vi "OnTrak_ADU_Write.vi"(2 "iTimeout":u32=200, 3 "Set Relay":i32=4 min=0 max=4 step=1, 4 "Output":u8 step=1 format="%x", 5 "psSerialNumber":string="E06002") -> (0 "OutPutNumber":i32 format="%x", 1 "error out":errorcluster)   [LabVIEW 2013]
uses:
  AduHid.dll
panel:
  out "OutPutStr":string="PK"
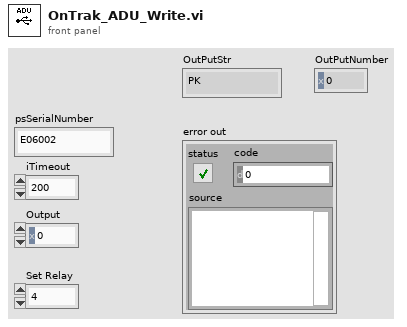
[diagram p1: front panel]
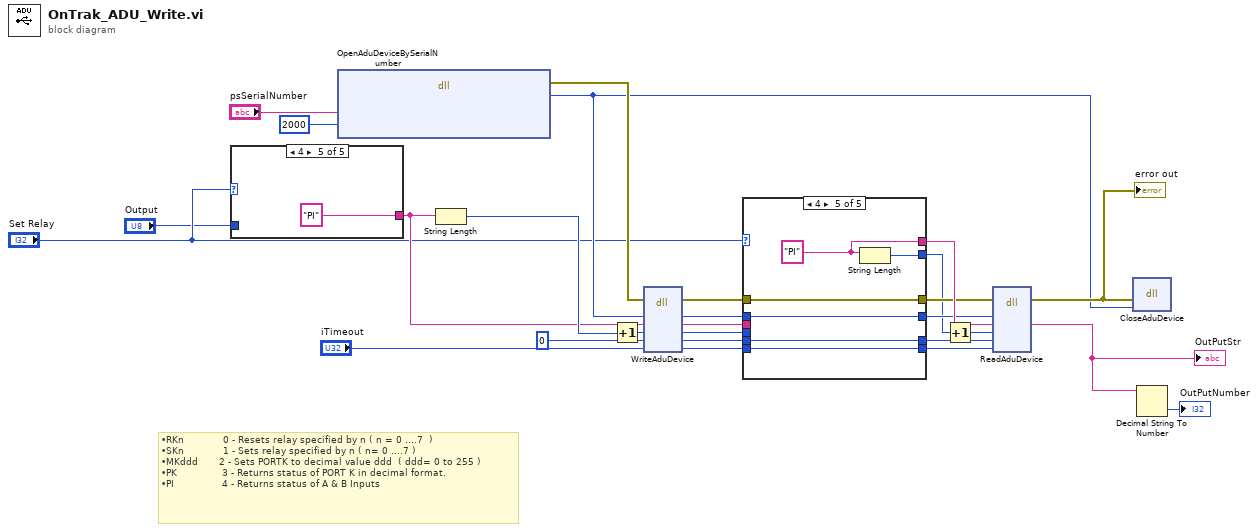
[diagram p0: block diagram]
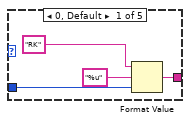
[diagram p2: hidden frame]
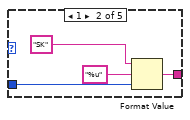
[diagram p3: hidden frame]
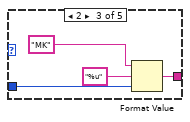
[diagram p4: hidden frame]
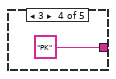
[diagram p5: hidden frame]
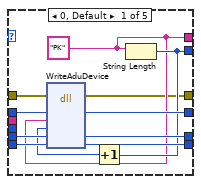
[diagram p6: hidden frame]
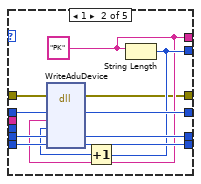
[diagram p7: hidden frame]
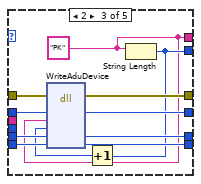
[diagram p8: hidden frame]
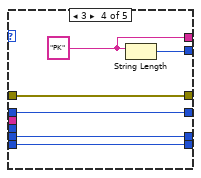
[diagram p9: hidden frame]
diagram:
  # "•RKn             0 - Resets relay specified by n ( n = 0 ....7  ) \n•SKn             1 - Sets relay specified by n ( n= 0 ....7 )\n•MKddd       2 - Sets PORTK to decimal value ddd  ( ddd= 0 to 255 )\n•PK               3 - Returns status of PORT K in decimal format.\n•PI                4 - Returns status of A & B Inputs"
  n1 = case shown="4" "Set Relay" {
    tunnel: [w30 w34 w38 "PK" "PI"] -> w21
    tunnel: "Output" -> [w29 w33 w37 _ _]
    frame 0, Default {
      n2 = Format Value(string ("")="RK", format string="%u", value (0)=w29) -> (output string=w30:string)
    }
    frame 1 {
      n3 = Format Value(string ("")="SK", format string="%u", value (0)=w33) -> (output string=w34:string)
    }
    frame 2 {
      n4 = Format Value(string ("")="MK", format string="%u", value (0)=w37) -> (output string=w38:string)
    }
    frame 3 {
    }
    frame 4 {
    }
  }
  n5 = dll-call lib="AduHid.dll" fn="OpenAduDeviceBySerialNumber"("psSerialNumber"="psSerialNumber", "iTimeout"=u32 2000) -> (error out=w26:errorcluster, "return type"=w25:u32)  [unwired: 5 in, 1 out]
  n6 = String Length(string=w21) -> (length=w24:i32)
  n7 = Increment(x=w24) -> (x+1=w2:i32)
  n8 = dll-call lib="AduHid.dll" fn="WriteAduDevice"(error in=w26, "aduHandle"=w25, "lpBuffer"=w21, "nNumberOfBytesToWrite"=w2, "lpNumberOfBytesWritten"=u32 0, "iTimeout"="iTimeout") -> (error out=w11:errorcluster, "aduHandle"=w18:u32, "lpBuffer"=w15:string, "nNumberOfBytesToWrite"=w14:u32, "lpNumberOfBytesWritten"=w17:u32, "iTimeout"=w16:u32)  [unwired: 3 in, 1 out]
  n9 = case shown="4" "Set Relay" {
    tunnel: [w46 w57 w66 w80 w86] -> w4
    tunnel: [w45 w56 w65 w79 w85] -> w22
    tunnel: w18 -> [w52 w61 w72 w76 w82]
    tunnel: w17 -> [w51 w62 w73 w77 w83]
    tunnel: w16 -> [w50 w63 w74 w78 w84]
    tunnel: w15 -> [_ _ _ _ _]
    tunnel: w14 -> [_ _ _ _ _]
    tunnel: [w49 w60 w71 w78 w84] -> w13
    tunnel: [w48 w59 w70 w77 w83] -> w1
    tunnel: [w47 w58 w69 w76 w82] -> w12
    tunnel: w11 -> [w44 w55 w68 w75 w81]
    tunnel: [w43 w54 w67 w75 w81] -> w10
    frame 0, Default {
      w45 = "PK"
      n10 = String Length(string=w45) -> (length=w46:i32)
      n11 = Increment(x=w46) -> (x+1=w42:i32)
      n12 = dll-call lib="AduHid.dll" fn="WriteAduDevice"(error in=w44, "aduHandle"=w52, "lpBuffer"=w45, "nNumberOfBytesToWrite"=w42, "lpNumberOfBytesWritten"=w51, "iTimeout"=w50) -> (error out=w43:errorcluster, "aduHandle"=w47:u32, "lpNumberOfBytesWritten"=w48:u32, "iTimeout"=w49:u32)  [unwired: 5 in, 1 out]
    }
    frame 1 {
      w56 = "PK"
      n13 = String Length(string=w56) -> (length=w57:i32)
      n14 = Increment(x=w57) -> (x+1=w53:i32)
      n15 = dll-call lib="AduHid.dll" fn="WriteAduDevice"(error in=w55, "aduHandle"=w61, "lpBuffer"=w56, "nNumberOfBytesToWrite"=w53, "lpNumberOfBytesWritten"=w62, "iTimeout"=w63) -> (error out=w54:errorcluster, "aduHandle"=w58:u32, "lpNumberOfBytesWritten"=w59:u32, "iTimeout"=w60:u32)  [unwired: 5 in, 1 out]
    }
    frame 2 {
      w65 = "PK"
      n16 = String Length(string=w65) -> (length=w66:i32)
      n17 = Increment(x=w66) -> (x+1=w64:i32)
      n18 = dll-call lib="AduHid.dll" fn="WriteAduDevice"(error in=w68, "aduHandle"=w72, "lpBuffer"=w65, "nNumberOfBytesToWrite"=w64, "lpNumberOfBytesWritten"=w73, "iTimeout"=w74) -> (error out=w67:errorcluster, "aduHandle"=w69:u32, "lpNumberOfBytesWritten"=w70:u32, "iTimeout"=w71:u32)  [unwired: 5 in, 1 out]
    }
    frame 3 {
      w79 = "PK"
      n19 = String Length(string=w79) -> (length=w80:i32)
    }
    frame 4 {
      w85 = "PI"
      n20 = String Length(string=w85) -> (length=w86:i32)
    }
  }
  n21 = Increment(x=w4) -> (x+1=w3:i32)
  n22 = dll-call lib="AduHid.dll" fn="ReadAduDevice"(error in=w10, "aduHandle"=w12, "lpBuffer"=w22, "nNumberOfBytesToWrite"=w3, "lpNumberOfBytesWritten"=w1, "iTimeout"=w13) -> (error out=w27:errorcluster, "lpBuffer"=w20:string)  [unwired: 7 in, 1 out]
  "error out" <- w27
  "OutPutStr" <- w20
  n23 = dll-call lib="AduHid.dll" fn="CloseAduDevice"(error in=w27, "hDevice"=w25) -> ()  [unwired: 4 in, 2 out]
  n24 = Decimal String To Number(string=w20) -> (number=→"OutPutNumber":i32)  [unwired: 2 in, 1 out]
